vi "VIH Project - Container - Group Rules.vi"(6 "cmd (get)":T9(ring), 8 "error in":errorcluster, 9 "Group Rule":T1, 10 "Group Idx (-1)":i32=-1, 11 "Group ID":string) -> (0 "error out":errorcluster, 1 "Group Rule out":T1, 2 "Group Idx out":i32, 3 "Group ID out":string, 5 "Group IDs":string[](array[string]))   [LabVIEW 2014]
doc: "::: VI Helpeks :::\nCopyright (c) 2000-2026 Konstantin Shifershteyn. All rights reserved."
uses:
  _VIH HelpGen.llb/VIH HelpGen Typedef - Cluster - Group Rule.ctl
  _VIH HelpGen.llb/VIH HelpGen Typedef - Enum - Default,Enable,Disable.ctl
  _VIH HelpGen.llb/VIH HelpGen Typedef - Cluster - Group Rule - Source Paths.ctl
  _VIH HelpGen.llb/VIH HelpGen Typedef - Cluster - Group Rule - Target Paths.ctl
  _VIH HelpGen.llb/VIH HelpGen Typedef - Enum - Description Mode.ctl
  _VIH HelpGen.llb/VIH HelpGen Typedef - Cluster - Control Rule.ctl
  _VIH HelpGen.llb/VIH HelpGen Typedef - Cluster - Enum Value Info.ctl
  _VIH HelpGen.llb/VIH HelpGen Typedef - Cluster - Group Rule - Flags.ctl
panel:
  # "VI Helpeks\nCopyright (c) 2012-2026 Konstantin Shifershteyn"
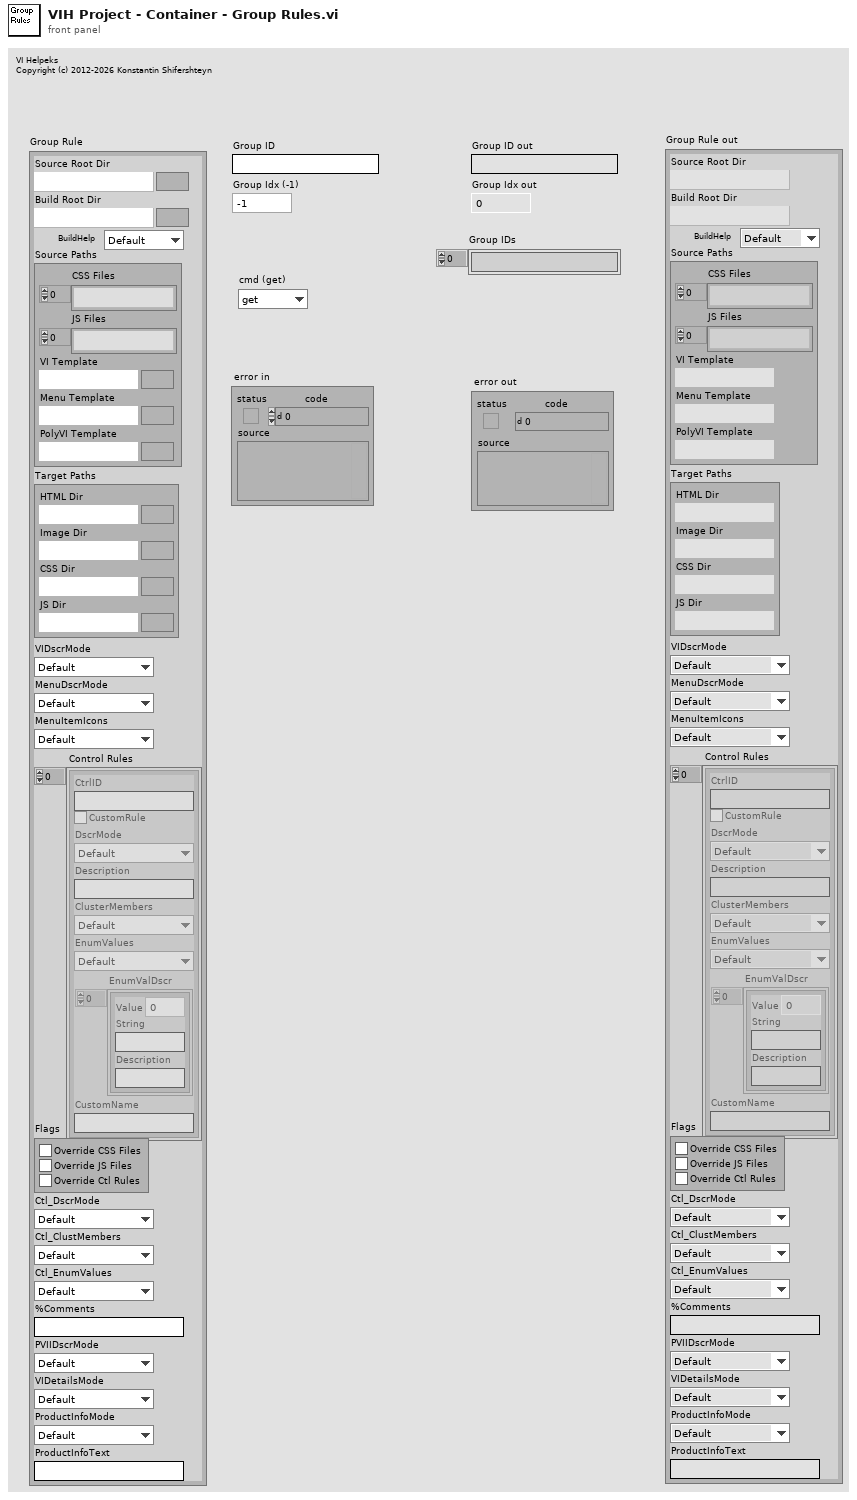
[diagram p1: front panel]
types:
  T1 = typedef "VIH HelpGen Typedef - Cluster - Group Rule.ctl" = cluster{"Source Root Dir":path, "Build Root Dir":path, "BuildHelp":T2, "Source Paths":T3, "Target Paths":T4, "VIDscrMode":T5, "MenuDscrMode":T5, "MenuItemIcons":T2, "Control Rules":T6[], "Flags":T8, "Ctl_DscrMode":T5, "Ctl_ClustMembers":T2, "Ctl_EnumValues":T2, "%Comments":string, "PVIIDscrMode":T5, "VIDetailsMode":T5, "ProductInfoMode":T2, "ProductInfoText":string}
  T2 = typedef "VIH HelpGen Typedef - Enum - Default,Enable,Disable.ctl" = enum16{"Default", "Enable", "Disable"}
  T3 = typedef "VIH HelpGen Typedef - Cluster - Group Rule - Source Paths.ctl" = cluster{"CSS Files":path[], "JS Files":path[], "VI Template":path, "Menu Template":path, "PolyVI Template":path}
  T4 = typedef "VIH HelpGen Typedef - Cluster - Group Rule - Target Paths.ctl" = cluster{"HTML Dir":path, "Image Dir":path, "CSS Dir":path, "JS Dir":path}
  T5 = typedef "VIH HelpGen Typedef - Enum - Description Mode.ctl" = enum16{"Default", "Description", "Description1", "Description2", "Custom", "None"}
  T6 = typedef "VIH HelpGen Typedef - Cluster - Control Rule.ctl" = cluster{"CtrlID":string, "CustomRule":bool, "DscrMode":T5, "Description":string, "ClusterMembers":T2, "EnumValues":T2, "EnumValDscr":T7[], "CustomName":string}
  T7 = typedef "VIH HelpGen Typedef - Cluster - Enum Value Info.ctl" = cluster{"Value":ext, "String":string, "Description":string}
  T8 = typedef "VIH HelpGen Typedef - Cluster - Group Rule - Flags.ctl" = cluster{"Override CSS Files":bool, "Override JS Files":bool, "Override Ctl Rules":bool}
  T9 = enum16{"get", "get all", "set", "Init", "delete"}
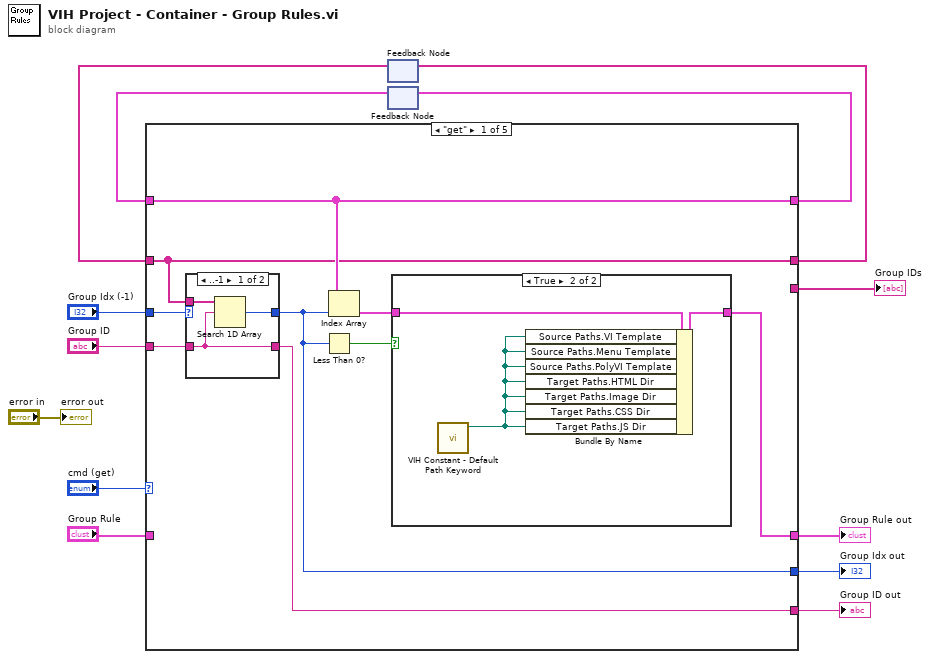
[diagram p0: block diagram]
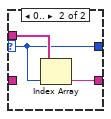
[diagram p3: hidden frame]
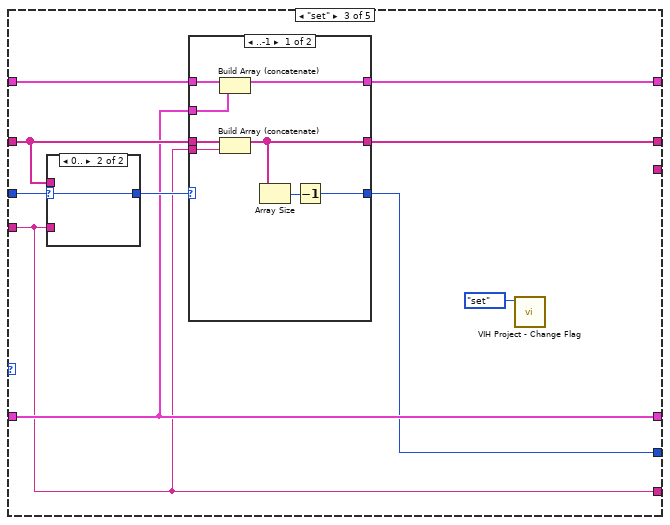
[diagram p5: hidden frame]
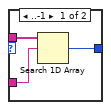
[diagram p6: hidden frame]
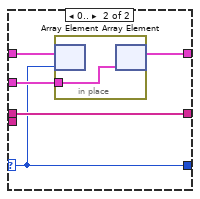
[diagram p7: hidden frame]
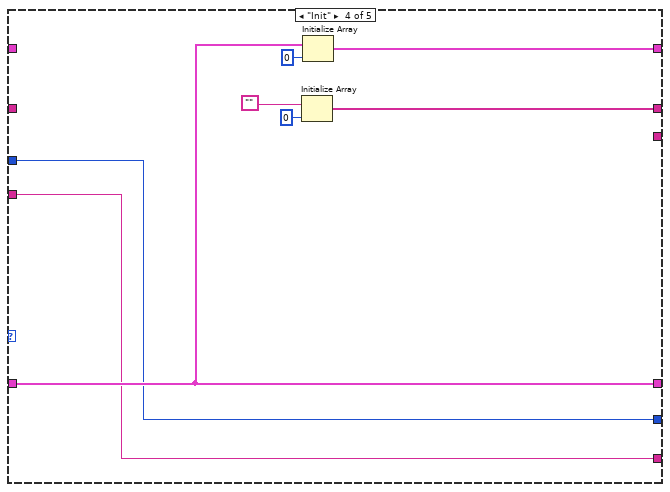
[diagram p8: hidden frame]
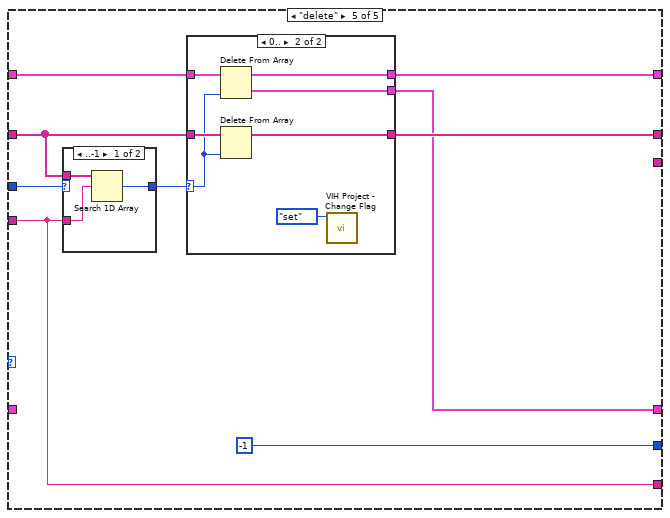
[diagram p9: hidden frame]
diagram:
  n1 = feedback #1() -> (w7:string[])  [unwired: 1 in]
  n2 = feedback #2() -> (w10:T1[])  [unwired: 1 in]
  n3 = case shown="\"get\"" "cmd (get)" {
    tunnel: "Group Rule" -> [_ w35 w41 w68 _]
    tunnel: [w22 w37 w46 w72 w81] -> w11
    tunnel: w10 -> [w22 w37 w47 _ w82]
    tunnel: [w20 w36 w45 w69 w80] -> w9
    tunnel: w7 -> [w20 w36 w43 _ w77]
    tunnel: [_ w36 _ _ _] -> w8
    tunnel: [w15 w35 w41 w68 w79] -> w6
    tunnel: "Group Idx (-1)" -> [w21 w34 w44 w67 w78]
    tunnel: "Group ID" -> [w19 w33 w39 w66 w74]
    tunnel: [w17 w34 w40 w67 -1 ("Item Idx (-1)")] -> w3
    tunnel: [w18 w33 w39 w66 w74] -> w2
    frame "get" {
      n4 = case shown="..-1" w21 {
        selector: w21 -> [_ w30]
        tunnel: [w29 w30] -> w17
        tunnel: w19 -> [w27 _]
        tunnel: w20 -> [w28 w31]
        tunnel: [w27 w32] -> w18
        frame ..-1 {
          n5 = Search 1D Array(1D array=w28, element=w27) -> (index of element=w29:i32)  [unwired: 1 in]
        }
        frame 0.. {
          n6 = Index Array(array=w31, index=w30) -> (element=w32:string)
        }
      }
      n7 = Less Than 0?(x=w17) -> (x < 0?=w16:bool)
      n8 = Index Array(array=w22, index=w17) -> (element=w14:T1)
      n9 = case shown="True" w16 {
        tunnel: [w23 w25] -> w15
        tunnel: w14 -> [w23 w26]
        frame False {
        }
        frame True {
          n10 = call "VIH Constant - Default Path Keyword.vi"() -> ("<default> path"=w24:path)  [unwired: 11 in]
          n11 = Bundle By Name(cluster=w26, "Source Paths.VI Template"=w24, "Source Paths.Menu Template"=w24, "Source Paths.PolyVI Template"=w24, "Target Paths.HTML Dir"=w24, "Target Paths.Image Dir"=w24, "Target Paths.CSS Dir"=w24, "Target Paths.JS Dir"=w24) -> (w25:T1)
        }
      }
    }
    frame "get all" {
    }
    frame "set" {
      n12 = case shown="0.." w44 {
        selector: w44 -> [_ w51]
        tunnel: [w50 w51] -> w42
        tunnel: w39 -> [w48 _]
        tunnel: w43 -> [w49 _]
        frame ..-1 {
          n13 = Search 1D Array(1D array=w49, element=w48) -> (index of element=w50:i32)  [unwired: 1 in]
        }
        frame 0.. {
        }
      }
      n14 = case shown="..-1" w42 {
        selector: w42 -> [_ w60]
        tunnel: w47 -> [w59 w64]
        tunnel: [w58 w63] -> w46
        tunnel: w43 -> [w57 w62]
        tunnel: [w52 w62] -> w45
        tunnel: w41 -> [w56 w61]
        tunnel: [w53 w60] -> w40
        tunnel: w39 -> [w55 _]
        frame ..-1 {
          n15 = Build Array (concatenate)(w59, w56) -> (w58:T1[])
          n16 = Build Array (concatenate)(w57, w55) -> (w52:string[])
          n17 = Array Size(array=w52) -> (size(s)=w54:i32)
          n18 = Decrement(x=w54) -> (x-1=w53:i32)
        }
        frame 0.. {
          n19 = in-place {
            in-place-border: w61 -> [w65]
            n20 = in-place-array #3(w64, w60) -> ()  [unwired: 1 out]
            n21 = in-place-array #3(w65) -> (w63:T1[])  [unwired: 1 out]
          }
        }
      }
      n22 = call "VIH Project - Change Flag.vi"("cmd (get)"=enum16{"get", "set", "reset"}."set") -> ()  [unwired: 9 in, 2 out]
    }
    frame "Init" {
      n23 = Initialize Array("", 0 ("dimension size")) -> (w69:string[])
      n24 = Initialize Array(w68, 0 ("dimension size")) -> (w72:T1[])
    }
    frame "delete" {
      n25 = case shown="..-1" w78 {
        selector: w78 -> [_ w86]
        tunnel: [w85 w86] -> w76
        tunnel: w74 -> [w83 _]
        tunnel: w77 -> [w84 _]
        frame ..-1 {
          n26 = Search 1D Array(1D array=w84, element=w83) -> (index of element=w85:i32)  [unwired: 1 in]
        }
        frame 0.. {
        }
      }
      n27 = case shown="0.." w76 {
        selector: w76 -> [_ w90]
        tunnel: w82 -> [w88 w95]
        tunnel: [w88 w94] -> w81
        tunnel: w77 -> [w87 w93]
        tunnel: [w87 w92] -> w80
        tunnel: [_ w91] -> w79
        frame ..-1 {
        }
        frame 0.. {
          n28 = Delete From Array(array=w95, index=w90) -> (deleted portion=w91:T1, array with subset deleted=w94:T1[])  [unwired: 1 in]
          n29 = Delete From Array(array=w93, index=w90) -> (array with subset deleted=w92:string[])  [unwired: 1 in, 1 out]
          n30 = call "VIH Project - Change Flag.vi"("cmd (get)"=enum16{"get", "set", "reset"}."set") -> ()  [unwired: 9 in, 2 out]
        }
      }
    }
  }
  "Group ID out" <- w2
  "Group Rule out" <- w6
  "Group IDs" <- w8
  "Group Idx out" <- w3
  n31 = feedback-in #1(w9) -> ()
  n32 = feedback-in #2(w11) -> ()
  "error out" <- "error in"
